vi "Create Messages For Registration.vi"(8 "error in (no error)":errorcluster, 10 "Messages MetaData":T1[](array[typedef]), 11 "VI in":refnum<vi>) -> (0 "error out":errorcluster, 3 "VI out":refnum<vi>)   [LabVIEW 2019, in "gRPC Template Creation Utility.lvlib"]
uses:
  gRPC Template Creation Utility.lvlib
  TypeDefs/Message Metadata (Scripting).ctl
  TypeDefs/Message Element Metadata (Scripting).ctl
  TypeDefs/Message Element Type.ctl
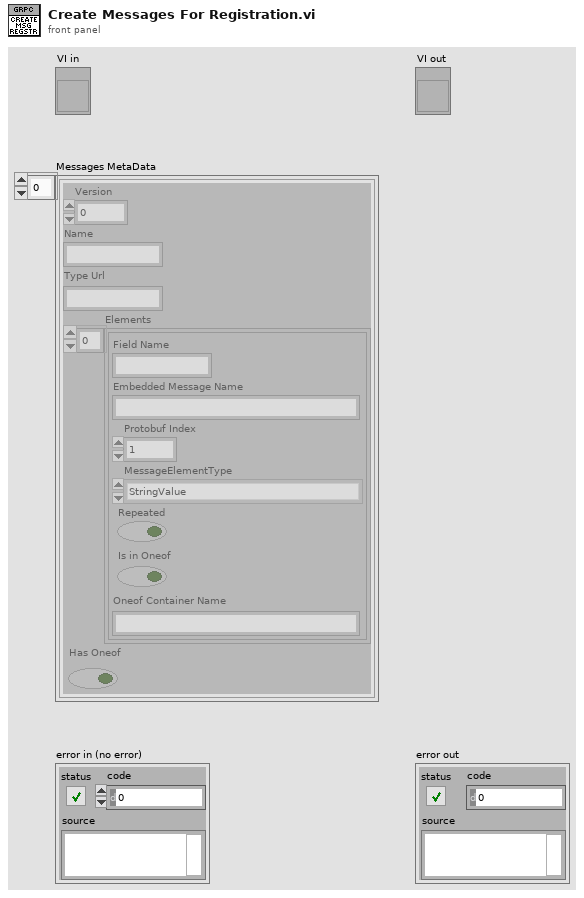
[diagram p1: front panel]
types:
  T1 = typedef "gRPC Template Creation Utility.lvlib/Message Metadata (Scripting).ctl" = cluster{"Version":i32, "Name":string, "Type Url":string, "Elements":T2[], "Has Oneof":bool}
  T2 = typedef "gRPC Template Creation Utility.lvlib/Message Element Metadata (Scripting).ctl" = cluster{"Field Name":string, "Embedded Message Name":string, "Protobuf Index":i32, "MessageElementType":T3, "Repeated":bool, "Is in Oneof":bool, "Oneof Container Name":string}
  T3 = typedef "gRPC Template Creation Utility.lvlib/Message Element Type.ctl" = enum32{"Int32Value", "FloatValue", "DoubleValue", "BoolValue", "StringValue", "MessageValue", "Int64Value", "UInt32Value", "UInt64Value", "EnumValue", "Bytes", "Fixed64", "Fixed32", "SFixed64", "SFixed32", "SInt64", "SInt32"}
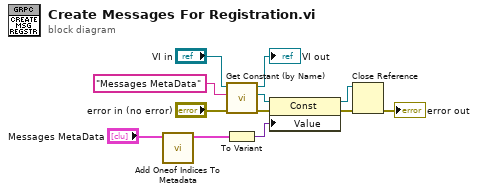
[diagram p0: block diagram]
diagram:
  n1 = call "Add Oneof Indices To Metadata.vi"("Messages MetaData"="Messages MetaData") -> ("Messages Metadata With Oneof Indices"=w2:T1[])  [unwired: 10 in]
  n2 = call "Get Constant (by Name).vi"("error in (no error)"="error in (no error)", "Constant Label"="Messages MetaData", "Owner VI in"="VI in") -> ("error out"=w7:errorcluster, "Const ref out"=w10:refnum<vi>, "Owner VI out"=→"VI out":refnum<vi>)  [unwired: 5 in, 1 out]
  n3 = To Variant(anything=w2) -> (Variant=w6:variant)
  n4 = property class="Const"(reference=w10, error in=w7, "Value"=w6) -> (reference out=w5:refnum<vi>, error out=w4:errorcluster)
  n5 = Close Reference(reference=w5, error in (no error)=w4) -> (error out=→"error out":errorcluster)
